vi "optical_get_image2.vi"() -> ()   [LabVIEW 2025]
uses:
  <vilib>/vision/driver/NI_Vision_Acquisition_Software.lvlib
  <vilib>/vision/driver/IMAQdx.llb/IMAQdx Acquisition Mode.ctl
  <vilib>/vision/driver/IMAQdx.llb/IMAQdx Buffer Number Mode.ctl
panel:
  out "Image":T1(plugin-control)
  out "error out":errorcluster
  out "Times between Frames":u32
  in  "Output Folder":path
  in  "Stop":bool
  in  "Camera Name":refnum<k21> caption="IMAQdx Session"
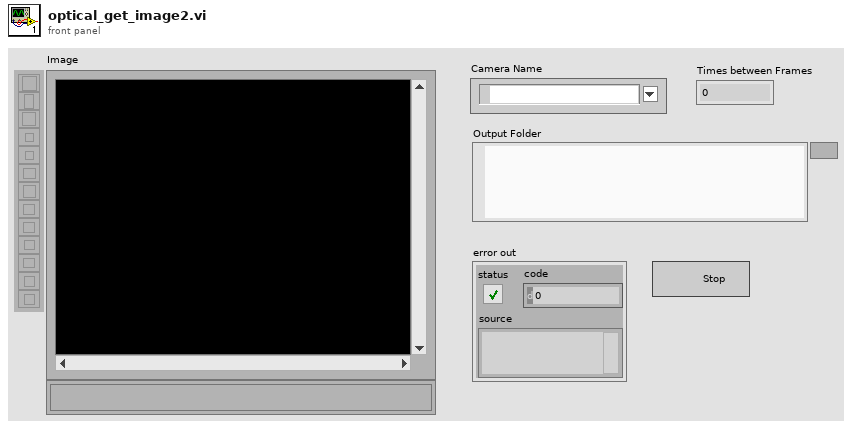
[diagram p1: front panel]
types:
  T1 = typedef "IMAQ Image.ctl" = refnum<image>
  T2 = typedef "Image Type" = u32
  T3 = typedef "NI_Vision_Acquisition_Software.lvlib/IMAQdx Acquisition Mode.ctl" = enum32{"One Shot", "Continuous"}
  T4 = typedef "IMAQdx.ctl" = refnum<k21>
  T5 = typedef "NI_Vision_Acquisition_Software.lvlib/IMAQdx Buffer Number Mode.ctl" = enum32{"Next", "Last", "Buffer Number", "Every", "Last New"}
  T6 = enum16{"big-endian, network order", "native, host order", "little-endian"}
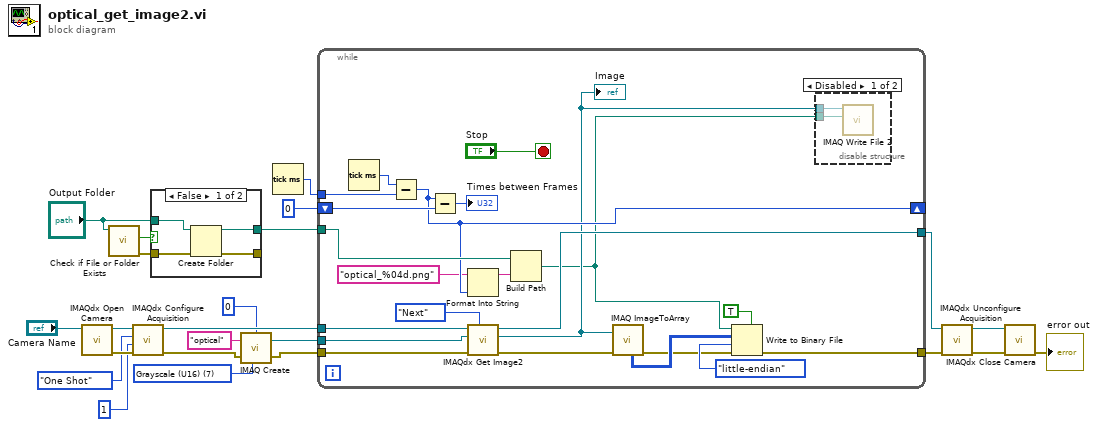
[diagram p0: block diagram]
diagram:
  w3 = T2 7 items=["Grayscale (U8)", "Grayscale (I16)", "Grayscale (SGL)", "Complex (CSG)", "RGB (U32)", "HSL (U32)", "RGB (U64)", "Grayscale (U16)"] ("Image Type")
  n1 = call <vilib>:"IMAQdx Open Camera.vi"("Session In"="Camera Name") -> ("error out"=w16:errorcluster, "Session Out"=w17:T4)  [unwired: 9 in]
  n2 = call <vilib>:"Check if File or Folder Exists.vi"("path"="Output Folder") -> ("error out"=w21:errorcluster, "file or folder exists?"=w23:bool)  [unwired: 8 in, 1 out]
  n3 = call <vilib>:"IMAQdx Configure Acquisition.vi"("error in"=w16, "Number of Buffers"=u32 1, "Continuous?"=IMAQdx_Acquisition_Mode."One Shot", "Session In"=w17) -> ("error out"=w5:errorcluster, "Session Out"=w11:T4)  [unwired: 6 in]
  n4 = case shown="False" w23 {
    tunnel: "Output Folder" -> [w27 w29]
    tunnel: [w26 w29] -> w20
    tunnel: w21 -> [w25 w28]
    tunnel: [w24 w28] -> _
    frame False {
      n5 = Create Folder(path (use dialog)=w27, error in=w25) -> (created path=w26:path, error out=w24:errorcluster)  [unwired: 1 in, 1 out]
    }
    frame True {
    }
  }
  n6 = call "IMAQ Create"("Border Size"=0, "Image Name"="optical", "Image Type"=w3, "error in (no error)"=w5) -> ("New Image"=w6:T1, "error out"=w4:errorcluster)  [unwired: 1 in]
  n7 = Tick Count (ms)() -> (millisecond timer value=w19:u32)
  n8 = while {
    tunnel: w20 -> [w51]
    tunnel: w19 -> [w49]
    shift-right: [w46] -> _
    shift-left: u32 0 -> [w47]
    tunnel: w11 -> [w41]
    tunnel: [w42] -> w10
    tunnel: [w33] -> w8
    tunnel: w4 -> [w40]
    tunnel: w6 -> [w31]
    stop <- "Stop" stop-if-true
    n9 = Tick Count (ms)() -> (millisecond timer value=w50:u32)
    n10 = Subtract(x=w50, y=w49) -> (x-y=w46:u32)
    n11 = Subtract(x=w46, y=w47) -> (x-y=→"Times between Frames":u32)
    n12 = Format Into String(format string="optical_%04d.png", w46) -> (resulting string=w45:string)  [unwired: 2 in, 1 out]
    n13 = call <vilib>:"IMAQdx Get Image2.vi"("Buffer Number Mode (Next)"=IMAQdx_Buffer_Number_Mode."Next", "error in"=w40, "Image In"=w31, "Session In"=w41) -> ("error out"=w32:errorcluster, "Image Out"=w36:T1, "Session Out"=w42:T4)  [unwired: 4 in, 1 out]
    "Image" <- w36
    n14 = Build Path(base path=w51, name or relative path=w45) -> (appended path=w35:path)
    n15 = call "IMAQ ImageToArray"("error in (no error)"=w32, "Image"=w36) -> ("Image Pixels (U16)"=w37:u16[][], "error out"=w34:errorcluster)  [unwired: 2 in, 3 out]
    n16 = Write to Binary File(file (use dialog)=w35, data=w37, error in=w34, 5:TRUE ("prepend array or string size? (T)"), 9:T6."little-endian" ("byte order (0:big-endian, network order)")) -> (error out=w33:errorcluster)  [unwired: 1 in, 2 out]
    n17 = disable-structure shown="Disabled" {
      disable-tunnel: w36 -> [w53 _]
      disable-tunnel: w35 -> [w52 _]
      frame Disabled {
        n18 = call-poly "IMAQ Write File 2"("File Path"=w52, "Image"=w53) -> ()  [unwired: 8 in, 2 out]
      }
      frame Enabled {
      }
    }
  }
  n19 = call <vilib>:"IMAQdx Unconfigure Acquisition.vi"("error in"=w8, "Session In"=w10) -> ("error out"=w7:errorcluster, "Session Out"=w9:T4)  [unwired: 8 in]
  n20 = call <vilib>:"IMAQdx Close Camera.vi"("error in"=w7, "Session In"=w9) -> ("error out"=→"error out":errorcluster)  [unwired: 9 in]
